vi "ALL - CE Examples.vi"   [LabVIEW 2021]
doc: "::: CalcExpress Toolkit :::\nCopyright (c) 2000-2026 Konstantin Shifershteyn. All rights reserved."
uses:
  cetypes.llb/CalcExpress Instance RefNum.ctl
types:
  T1 = typedef "CalcExpress Instance RefNum.ctl" = refnum<k1>
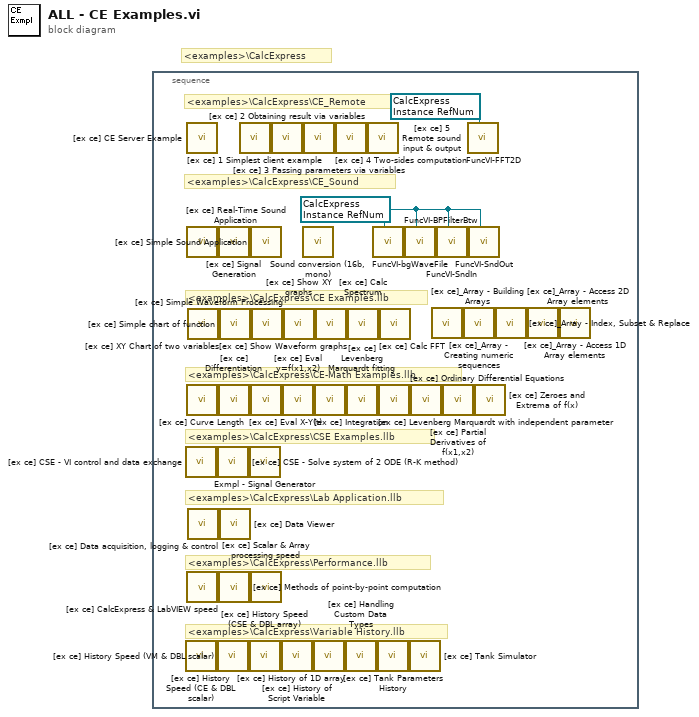
[diagram p0: block diagram]
diagram:
  # "<examples>\\CalcExpress"
  n1 = stacked-sequence {
    frame #0 {
      w1 = T1 refnum items=["CE RefNum"] ("InstanceRef")
      w2 = T1 refnum items=["CE RefNum"] ("InstanceRef")
      # "<examples>\\CalcExpress\\Variable History.llb"
      # "<examples>\\CalcExpress\\Performance.llb"
      # "<examples>\\CalcExpress\\Lab Application.llb"
      # "<examples>\\CalcExpress\\CSE Examples.llb"
      # "<examples>\\CalcExpress\\CE-Math Examples.llb"
      # "<examples>\\CalcExpress\\CE Examples.llb"
      # "<examples>\\CalcExpress\\CE_Sound"
      # "<examples>\\CalcExpress\\CE_Remote"
      n2 = call "[ex ce] CSE - VI control and data exchange.vi"() -> ()  [unwired: 1 in]
      n3 = call "[ex ce] History Speed (CE & DBL scalar).vi"() -> ()  [unwired: 1 in]
      n4 = call "[ex ce] CE Server Example.vi"() -> ()  [unwired: 1 in]
      n5 = call "[ex ce] Real-Time Sound Application.vi"() -> ()  [unwired: 1 in]
      n6 = call "[ex ce] Curve Length.vi"() -> ()  [unwired: 1 in]
      n7 = call "[ex ce] CalcExpress & LabVIEW speed.vi"() -> ()  [unwired: 7 in]
      n8 = call "[ex ce] XY Chart of two variables.vi"() -> ()  [unwired: 12 in]
      n9 = call "[ex ce] Data acquisition, logging & control.vi"() -> ()  [unwired: 1 in]
      n10 = call "[ex ce] CSE - Solve system of 2 ODE (R-K method).vi"() -> ()  [unwired: 1 in]
      n11 = call "[ex ce] History Speed (VM & DBL scalar).vi"() -> ()  [unwired: 1 in]
      n12 = call "[ex ce] Signal Generation.vi"() -> ()  [unwired: 1 in]
      n13 = call "[ex ce] Differentiation.vi"() -> ()  [unwired: 1 in]
      n14 = call "[ex ce] Methods of point-by-point computation.vi"() -> ()  [unwired: 1 in]
      n15 = call "[ex ce] Simple chart of function.vi"() -> ()  [unwired: 12 in]
      n16 = call "[ex ce] Data Viewer.vi"() -> ()  [unwired: 1 in]
      n17 = call "[ex ce] 1 Simplest client example.vi"() -> ()  [unwired: 1 in]
      n18 = call "Exmpl - Signal Generator.vi"() -> ()  [unwired: 1 in]
      n19 = call "[ex ce] History Speed (CSE & DBL array).vi"() -> ()  [unwired: 1 in]
      n20 = call "[ex ce] Simple Sound Application.vi"() -> ()  [unwired: 1 in]
      n21 = call "[ex ce] Eval X-Y(t).vi"() -> ()  [unwired: 1 in]
      n22 = call "[ex ce] Scalar & Array processing speed.vi"() -> ()  [unwired: 7 in]
      n23 = call "[ex ce] Simple Waveform Processing.vi"() -> ()  [unwired: 1 in]
      n24 = call "[ex ce] 2 Obtaining result via variables.vi"() -> ()  [unwired: 1 in]
      n25 = call "[ex ce] History of Script Variable.vi"() -> ()  [unwired: 1 in]
      n26 = call "[ex ce] Eval y=f(x1,x2).vi"() -> ()  [unwired: 1 in]
      n27 = call "[ex ce] Show XY graphs.vi"() -> ()  [unwired: 12 in]
      n28 = call "Sound conversion (16b, mono).vi"() -> ()  [unwired: 10 in, 2 out]
      n29 = call "[ex ce] 3 Passing parameters via variables.vi"() -> ()  [unwired: 1 in]
      n30 = call "[ex ce] History of 1D array.vi"() -> ()  [unwired: 1 in]
      n31 = call "[ex ce] Integration.vi"() -> ()  [unwired: 1 in]
      n32 = call "[ex ce] Show Waveform graphs.vi"() -> ()  [unwired: 12 in]
      n33 = call "[ex ce] 4 Two-sides computation.vi"() -> ()  [unwired: 1 in]
      n34 = call "[ex ce] Handling Custom Data Types.vi"() -> ()  [unwired: 1 in]
      n35 = call "[ex ce] Levenberg Marquardt fitting.vi"() -> ()  [unwired: 1 in]
      n36 = call "[ex ce] Calc Spectrum.vi"() -> ()  [unwired: 12 in]
      n37 = call "[ex ce] 5 Remote sound input & output.vi"() -> ()  [unwired: 1 in]
      n38 = call "FuncVI-bgWaveFile.vi"("InstanceRef"=w1) -> ()  [unwired: 7 in, 2 out]
      n39 = call "[ex ce] Tank Parameters History.vi"() -> ()  [unwired: 1 in]
      n40 = call "[ex ce] Levenberg Marquardt with independent parameter.vi"() -> ()  [unwired: 1 in]
      n41 = call "[ex ce] Calc FFT.vi"() -> ()  [unwired: 12 in]
      n42 = call "FuncVI-BPFilterBtw.vi"("InstanceRef"=w1) -> ()  [unwired: 7 in, 2 out]
      n43 = call "[ex ce] Tank Simulator.vi"() -> ()  [unwired: 1 in]
      n44 = call "[ex ce] Ordinary Differential Equations.vi"() -> ()  [unwired: 11 in, 1 out]
      n45 = call "[ex ce]_Array - Building Arrays.vi"() -> ()  [unwired: 12 in]
      n46 = call "FuncVI-SndIn.vi"("InstanceRef"=w1) -> ()  [unwired: 7 in, 2 out]
      n47 = call "[ex ce] Partial Derivatives of f(x1,x2).vi"() -> ()  [unwired: 1 in]
      n48 = call "[ex ce]_Array - Creating numeric sequences.vi"() -> ()  [unwired: 12 in]
      n49 = call "FuncVI-FFT2D.vi"("InstanceRef"=w2) -> ()  [unwired: 7 in, 2 out]
      n50 = call "FuncVI-SndOut.vi"("InstanceRef"=w1) -> ()  [unwired: 7 in, 2 out]
      n51 = call "[ex ce] Zeroes and Extrema of f(x) .vi"() -> ()  [unwired: 1 in]
      n52 = call "[ex ce]_Array - Index, Subset & Replace.vi"() -> ()  [unwired: 1 in]
      n53 = call "[ex ce]_Array - Access 2D Array elements.vi"() -> ()  [unwired: 12 in]
      n54 = call "[ex ce]_Array - Access 1D Array elements.vi"() -> ()  [unwired: 12 in]
    }
  }
